vi "02_ui_smith_plot.vi"() -> ()   [LabVIEW 2025]
uses:
  213d4d69-42c2-4ab9-8e5c-f09799411473.vi
  9924c898-3be5-4834-b900-de0bc968c1de.vi
  9ab8033c-be5d-4a17-bbd5-1ebfae571c10.vi
panel:
  out "r_norm":dbl caption="Cursor - R"
  out "jx_norm":dbl caption="Cursor - jX"
  out "phase_cursor":dbl caption="Phase"
  out "jx_cursor":dbl caption="jX"
  out "r_cursor":dbl caption="R"
  out "smith_dimensions":i16
  out "frequency_cursor":string caption="Frequency"
  out "panel_resized":bool=TRUE
  out "smith_plot":picture
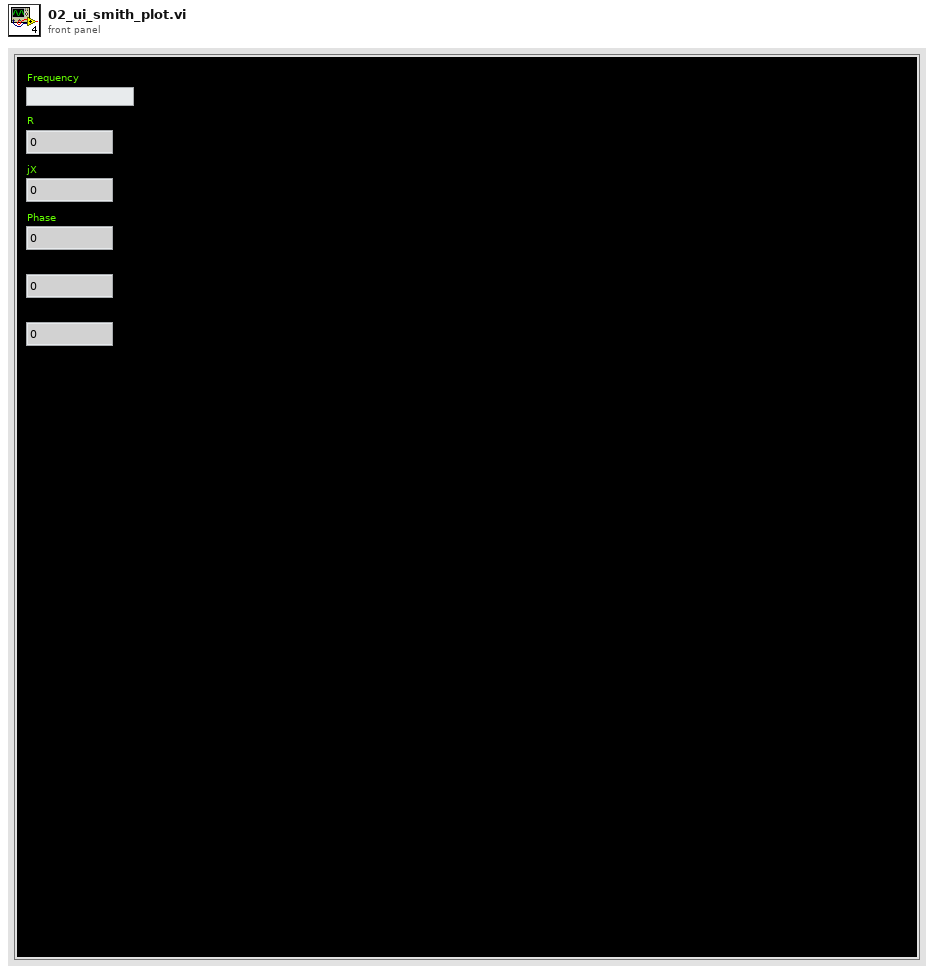
[diagram p1: front panel]
types:
  T1 = cluster{"button_load_sxp":bool, "button_load_csv":bool, "button_save_s1p":bool, "button_save_s2p":bool, "button_single_sweep":bool, "tcp_load_cal":bool, "show_smith_window":bool}
  T2 = cluster{"freq_array":dbl[], "data_array":dbl[]}[]
  T3 = typedef "LVRectTypeDef.ctl" = cluster{"Left":i16, "Top":i16, "Right":i16, "Bottom":i16}
  T4 = typedef "LVPoint32TypeDef.ctl" = cluster{"Horizontal":i32, "Vertical":i32}
  T5 = cluster{"frequency":dbl, "r":dbl, "jx":dbl, "phase":dbl}
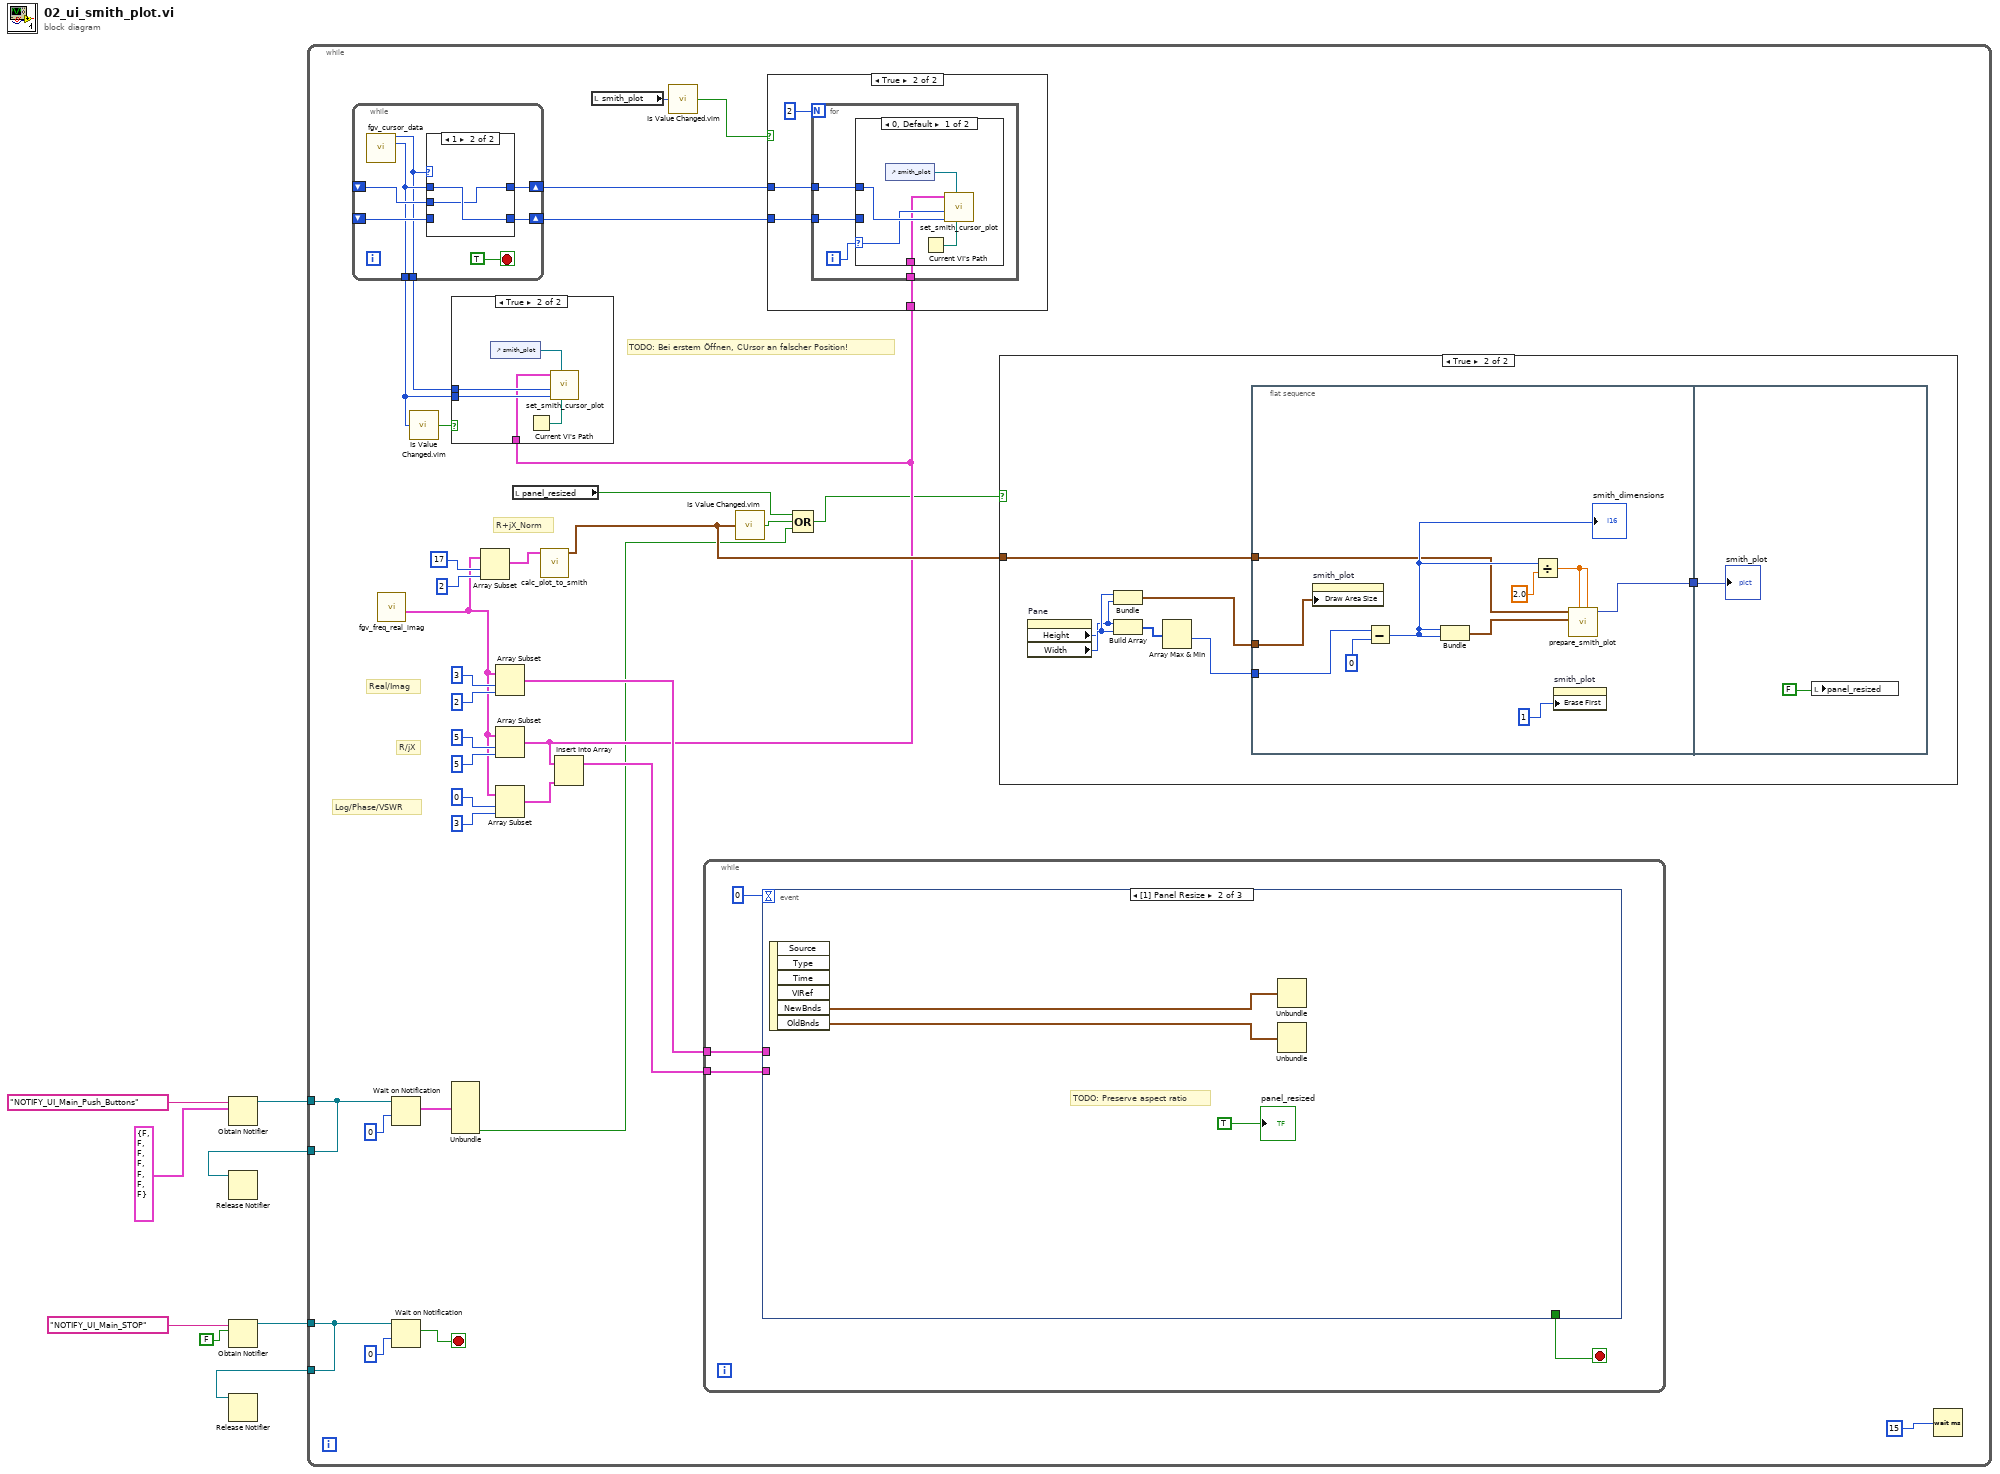
[diagram p0: block diagram]
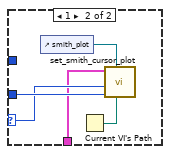
[diagram p4: hidden frame]
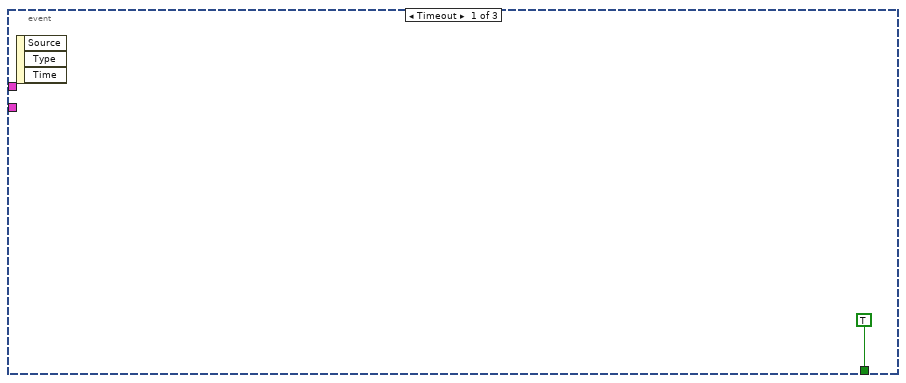
[diagram p6: hidden frame]
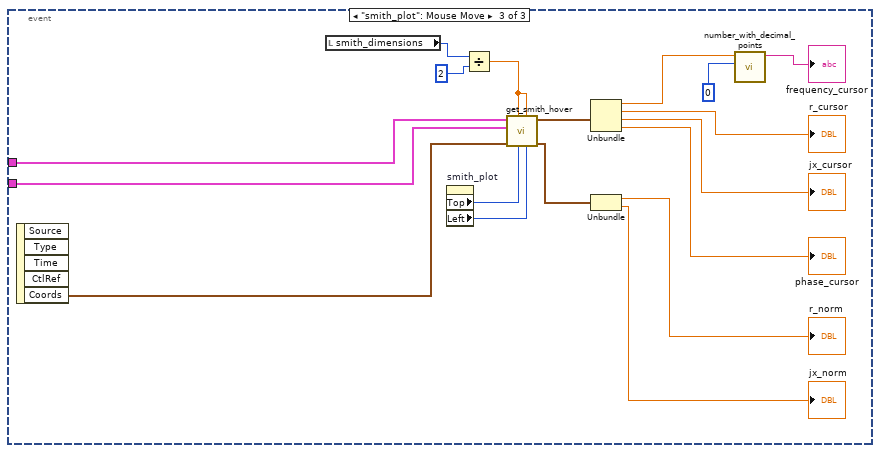
[diagram p7: hidden frame]
diagram:
  n1 = Obtain Notifier(name (unnamed)="NOTIFY_UI_Main_Push_Buttons", notification data type=T1 {"button_load_sxp"=FALSE, "button_load_csv"=FALSE, "button_save_s1p"=FALSE, "button_save_s2p"=FALSE, "button_single_sweep"=FALSE, "tcp_load_cal"=FALSE, "show_smith_window"=FALSE} ("output cluster")) -> (notifier out=w3:refnum<notifier>)  [unwired: 2 in, 2 out]
  n2 = Obtain Notifier(name (unnamed)="NOTIFY_UI_Main_STOP", notification data type=FALSE) -> (notifier out=w6:refnum<notifier>)  [unwired: 2 in, 2 out]
  n3 = while {
    tunnel: w6 -> [w39]
    tunnel: [w39] -> w5
    tunnel: w3 -> [w32]
    tunnel: [w32] -> w2
    stop <- w38 stop-if-true
    # "TODO: Bei erstem Öffnen, CUrsor an falscher Position!"
    # "Log/Phase/VSWR"
    # "R/jX"
    # "Real/Imag"
    # "R+jX_Norm"
    n4 = while {
      shift-right: [w70] -> w19
      shift-left: _ -> [w68]
      shift-right: [w69] -> w20
      shift-left: _ -> [w67]
      tunnel: [w66] -> w15
      tunnel: [w65] -> w18
      stop <- TRUE stop-if-true
      n5 = call "fgv_cursor_data.vi"() -> ("cursor_idx_get"=w65:i32, "cursor_pos_get"=w66:i32)  [unwired: 9 in, 5 out]
      n6 = case shown="1" w65 {
        tunnel: w66 -> [w73 w75]
        tunnel: [w73 w74] -> w70
        tunnel: [w72 w75] -> w69
        tunnel: w68 -> [_ w74]
        tunnel: w67 -> [w72 _]
        frame 0, Default {
        }
        frame 1 {
        }
      }
    }
    n7 = call "fgv_freq_real_imag.vi"() -> ("plot_data"=w21:T2)  [unwired: 8 in, 3 out]
    n8 = Wait on Notification(notifier=w32, timeout in ms (-1)=0) -> (notification=w34:T1)  [unwired: 2 in, 3 out]
    n9 = Wait on Notification(notifier=w39, timeout in ms (-1)=0) -> (notification=w38:bool)  [unwired: 2 in, 3 out]
    n10 = call "Is Value Changed.vim"("value"=w15) -> ("changed or first call?"=w14:bool)
    n11 = Unbundle(w34) -> ("show_smith_window"=w9:bool)  [unwired: 6 out]
    n12 = Array Subset(array=w21, index=17, length=2) -> (w35:T2)
    n13 = Array Subset(array=w21, index=3, length=2) -> (w23:T2)
    n14 = Array Subset(array=w21, index=5, length=5) -> (w17:T2)
    n15 = case shown="True" w14 {
      tunnel: w15 -> [_ w44]
      tunnel: w18 -> [_ w43]
      tunnel: w17 -> [_ w42]
      frame False {
      }
      frame True {
        n16 = control-ref of="smith_plot"() -> (w45:refnum<vi>)
        n17 = Current VI's Path() -> (path=w46:path)
        n18 = call "set_smith_cursor_plot.vi"("path"=w46, "smith_plot"=w45, "cursor_pos"=w44, "cursor_index"=w43, "plot_rjx"=w42) -> ()  [unwired: 7 in]
      }
    }
    n19 = Array Subset(array=w21, index=0, length=3) -> (w25:T2)
    n20 = local read "panel_resized"() -> (w11:bool)
    n21 = call "calc_plot_to_smith.vi"("Plot_Data"=w35) -> ("smith plot"=w22:cluster{"r":dbl, "x":dbl}[])  [unwired: 10 in]
    n22 = Insert Into Array(array=w17, new element=w25) -> (w24:T2)  [unwired: 1 in]
    n23 = local read "smith_plot"() -> (w16:picture)
    n24 = call "Is Value Changed.vim"("value"=w16) -> ("changed or first call?"=w13:bool)
    n25 = while {
      tunnel: w24 -> [w77]
      tunnel: w23 -> [w76]
      stop <- w78 stop-if-true
      n26 = event shown="[1] Panel Resize" {
        selector: _ -> [_ _ _]
        dyn-events: _ -> [_ _ _]
        timeout: 0 -> [_ _ _]
        tunnel: [TRUE _ _] -> w78
        tunnel: w77 -> [_ _ w85]
        tunnel: w76 -> [_ _ w84]
        event Timeout {
          n27 = event-data() -> ()  [unwired: 1 in, 3 out]
        }
        event Panel Resize {
          # "TODO: Preserve aspect ratio"
          n28 = event-data() -> ("NewBnds"=w81:T3, "OldBnds"=w82:T3)  [unwired: 1 in, 4 out]
          n29 = Unbundle(w81) -> ()  [unwired: 4 out]
          n30 = Unbundle(w82) -> ()  [unwired: 4 out]
          "panel_resized" <- TRUE
        }
        event "smith_plot": Mouse Move {
          n31 = event-data() -> ("Coords"=w101:T4)  [unwired: 1 in, 4 out]
          n32 = local read "smith_dimensions"() -> (w96:i16)
          n33 = property on="smith_plot" class="Pict"() -> ("Top"=w99:i32, "Left"=w98:i32)  [unwired: 2 in, 2 out]
          n34 = Divide(x=w96, y=u32 2) -> (x/y=w94:dbl)
          n35 = call "get_smith_hover.vi"("smith_pos_left"=w98, "left_center"=w94, "smith_pos_top"=w99, "top_center"=w94, "Coords"=w101, "cursor_data"=w85, "ref_data"=w84) -> ("cursor_pos"=w88:cluster{"r_norm":dbl, "x_norm":dbl}, "cursor_data"=w93:T5)  [unwired: 3 in]
          n36 = Unbundle(w93) -> ("frequency"=w89:dbl, "r"=→"r_cursor":dbl, "jx"=→"jx_cursor":dbl, "phase"=→"phase_cursor":dbl)
          n37 = Unbundle(w88) -> ("r_norm"=→"r_norm":dbl, "x_norm"=→"jx_norm":dbl)
          n38 = call "number_with_decimal_points.vi"("Precision"=i16 0, "Double"=w89) -> ("String"=→"frequency_cursor":string)  [unwired: 5 in]
        }
      }
    }
    n39 = call "Is Value Changed.vim"("value"=w22) -> ("changed or first call?"=w12:bool)
    n40 = case shown="True" w13 {
      tunnel: w19 -> [_ w49]
      tunnel: w20 -> [_ w48]
      tunnel: w17 -> [_ w47]
      frame False {
      }
      frame True {
        n41 = for {
          N: 2 -> [_]
          tunnel: w49 -> [w53]
          tunnel: w48 -> [w52]
          tunnel: w47 -> [w51]
          i -> [w54]
          n42 = case shown="0, Default" w54 {
            selector: w54 -> [w56 w61]
            tunnel: w53 -> [w57 _]
            tunnel: w52 -> [_ w62]
            tunnel: w51 -> [w55 w60]
            frame 0, Default {
              n43 = control-ref of="smith_plot"() -> (w59:refnum<vi>)
              n44 = Current VI's Path() -> (path=w58:path)
              n45 = call "set_smith_cursor_plot.vi"("path"=w58, "smith_plot"=w59, "cursor_pos"=w57, "cursor_index"=w56, "plot_rjx"=w55) -> ()  [unwired: 7 in]
            }
            frame 1 {
              n46 = control-ref of="smith_plot"() -> (w64:refnum<vi>)
              n47 = Current VI's Path() -> (path=w63:path)
              n48 = call "set_smith_cursor_plot.vi"("path"=w63, "smith_plot"=w64, "cursor_pos"=w62, "cursor_index"=w61, "plot_rjx"=w60) -> ()  [unwired: 7 in]
            }
          }
        }
      }
    }
    n49 = Compound Arithmetic op=OR(w11, w12, w9) -> (w10:bool)
    n50 = case shown="True" w10 {
      tunnel: w22 -> [_ w103]
      frame False {
      }
      frame True {
        n51 = property on="Pane" class="Pane"() -> ("Height"=w106:u32, "Width"=w107:u32)  [unwired: 2 in, 2 out]
        n52 = Bundle("Width"=w107, "Height"=w106) -> (w105:cluster{"Width":u32, "Height":u32})  [unwired: 1 in]
        n53 = Build Array(w106, w107) -> (w108:u32[])
        n54 = Array Max & Min(array=w108) -> (min value=w102:u32)  [unwired: 3 out]
        n55 = flat-sequence {
          tunnel: w102 -> [w117]
          tunnel: w105 -> [w115]
          tunnel: [w110] -> w104
          tunnel: w103 -> [w109]
          tunnel: w104 -> [w119]
          frame #0 {
            n56 = property on="smith_plot" class="Pict"("Draw Area Size"=w115) -> ()  [unwired: 2 in, 2 out]
            n57 = Subtract(x=w117, y=u32 0) -> (x-y=w113:u32)
            "smith_dimensions" <- w113
            n58 = Bundle(w113, w113) -> (w112:cluster{u32, u32})  [unwired: 1 in]
            n59 = Divide(x=w113, y=2.0) -> (x/y=w111:dbl)
            n60 = property on="smith_plot" class="Pict"("Erase First"=u8 1) -> ()  [unwired: 2 in, 2 out]
            n61 = call "prepare_smith_plot.vi"("left_center"=w111, "top_center"=w111, "dimensions (w,h)"=w112, "smith plot"=w109) -> ("smith_out"=w110:picture)  [unwired: 7 in]
          }
          frame #1 {
            n62 = local write "panel_resized"(FALSE ("Boolean")) -> ()
            "smith_plot" <- w119
          }
        }
      }
    }
    n63 = Wait (ms)(milliseconds to wait=u32 15) -> ()  [unwired: 1 out]
  }
  n64 = Release Notifier(notifier=w2) -> ()  [unwired: 2 in, 3 out]
  n65 = Release Notifier(notifier=w5) -> ()  [unwired: 2 in, 3 out]
